vi "prueba_prueba.vi"() -> ()   [LabVIEW 2019]
uses:
  <vilib>/myRIO/Common/Instrument Driver Framework/myRIO v1.0/Encoder/typedefs/Encoder Signal Mode.ctl
  <vilib>/myRIO/Instrument Drivers/Onboard IO/Encoder/typedefs/Encoder Reference.ctl
  <vilib>/myRIO/Common/Instrument Driver Framework/Utilities/typedefs/myRIO Generic Hardware Reference.ctl
  <vilib>/myRIO/Common/Instrument Driver Framework/Utilities/typedefs/Hardware Version Enum.ctl
  <vilib>/myRIO/Common/Instrument Driver Framework/Utilities/typedefs/myRIO v1.0 Reference.ctl
  <vilib>/myRIO/Common/Instrument Driver Framework/Utilities/typedefs/Generic FPGA Reference.ctl
  <vilib>/myRIO/Common/Instrument Driver Framework/myRIO v1.0/Encoder/typedefs/Encoder Channels Enum.ctl
  <vilib>/myRIO/Common/Instrument Driver Framework/myRIO v1.0/Encoder/typedefs/Encoder Configuration v1.0.ctl
  <vilib>/userDefined/High Color/nirio_resource_hc.ctl
  <vilib>/myRIO/Instrument Drivers/Onboard IO/UART/typedef/VISA Configuration.ctl
  <vilib>/myRIO/Instrument Drivers/Onboard IO/DIO/typedefs/DIO Reference.ctl
  <vilib>/myRIO/Common/Instrument Driver Framework/myRIO v1.0/DIO/typedefs/DIO Channels List.ctl
  <vilib>/myRIO/Common/Instrument Driver Framework/myRIO v1.0/DIO/typedefs/DIO Channels Enum.ctl
  <vilib>/myRIO/Instrument Drivers/Onboard IO/PWM/typedefs/PWM Reference.ctl
  <vilib>/myRIO/Common/Instrument Driver Framework/myRIO v1.0/PWM/typedefs/PWM Channels Enum.ctl
  <vilib>/myRIO/Instrument Drivers/Onboard IO/PWM/typedefs/PWM Configuration.ctl
  <vilib>/myRIO/Common/Instrument Driver Framework/Utilities/vis/Is FPGA Ref Available.vi
  <vilib>/myRIO/Common/Instrument Driver Framework/myRIO v1.0/Encoder/vis/myRIO v1.1 Open Encoder.vi
  <vilib>/myRIO/Instrument Drivers/Onboard IO/Encoder/vis/Read.vi
  <vilib>/myRIO/Common/Instrument Driver Framework/myRIO v1.0/DIO/vis/myRIO v1.1 Open DIO.vi
  <vilib>/myRIO/Instrument Drivers/Onboard IO/DIO/vis/Write.vi
  <vilib>/myRIO/Common/Instrument Driver Framework/myRIO v1.0/PWM/vis/myRIO v1.1 Open PWM.vi
  <vilib>/myRIO/Instrument Drivers/Onboard IO/PWM/vis/Set Duty Cycle and Frequency.vi
  <vilib>/myRIO/Common/Instrument Driver Framework/Utilities/vis/Validate Channels.vi
  <vilib>/myRIO/Common/Instrument Driver Framework/myRIO v1.0/Encoder/vis/myRIO v1.0 Reserve Encoder.vi
  <vilib>/myRIO/Common/Instrument Driver Framework/myRIO v1.0/DIO/vis/myRIO v1.0 Reserve DIO.vi
  <vilib>/myRIO/Common/Instrument Driver Framework/myRIO v1.0/PWM/vis/myRIO v1.0 Reserve PWM.vi
  <vilib>/myRIO/Common/Instrument Driver Framework/myRIO v1.0/Encoder/vis/myRIO v1.0 Build MUX Configuration Encoder.vi
  <vilib>/myRIO/Common/Instrument Driver Framework/myRIO v1.0/Resource Manager/vis/myRIO v1.0 Reserve Channel List.vi
  <vilib>/myRIO/Common/Instrument Driver Framework/myRIO v1.0/DIO/vis/myRIO v1.0 Build MUX Configuration DIO.vi
  <vilib>/myRIO/Common/Instrument Driver Framework/myRIO v1.0/PWM/vis/myRIO v1.0 Build MUX Configuration PWM.vi
  <vilib>/myRIO/Common/Instrument Driver Framework/myRIO v1.0/Resource Manager/vis/myRIO v1.0 Create Configuration List.vi
  <vilib>/myRIO/Common/Instrument Driver Framework/myRIO v1.0/Resource Manager/vis/myRIO v1.0 Reserve Channel.vi
  <vilib>/myRIO/Common/Instrument Driver Framework/myRIO v1.0/Resource Manager/vis/myRIO v1.0 Unreserve Channel.vi
  <vilib>/myRIO/Common/Instrument Driver Framework/myRIO v1.0/Resource Manager/vis/myRIO v1.0 Build Mutex Name.vi
  <vilib>/Utility/VariantDataType/GetNumericInfo.vi
  <vilib>/Utility/error.llb/Error Cluster From Error Code.vi
  <vilib>/myRIO/Common/Instrument Driver Framework/myRIO v1.0/myRIO v1.1 Open.vi
  <vilib>/myRIO/Common/Instrument Driver Framework/Utilities/vis/IO Manager.vi
  <vilib>/myRIO/Common/Instrument Driver Framework/Utilities/vis/Configuration Manager.vi
  <vilib>/myRIO/Common/Instrument Driver Framework/myRIO v1.0/Resource Manager/vis/myRIO v1.0 Configure IO.vi
  <vilib>/myRIO/Common/Instrument Driver Framework/myRIO v1.0/myRIO v1.0 Close.vi
  <vilib>/myRIO/Common/Instrument Driver Framework/myRIO v1.0/Encoder/vis/myRIO v1.0 Configure Encoder.vi
  <vilib>/myRIO/Common/Instrument Driver Framework/myRIO v1.0/Encoder/vis/myRIO v1.0 Read Encoder.vi
  <vilib>/Instr/_visa.llb/VISA Configure Serial Port (Instr).vi
  <vilib>/express/express shared/transition.llb/Dynamic To Waveform Array.vi
  <vilib>/express/express signal manip/GetorSetDDTAttributes/Set DDT Attributes/SetT0.vi
  <vilib>/express/express shared/transition.llb/Waveform Array To Dynamic.vi
  <vilib>/myRIO/Common/Instrument Driver Framework/myRIO v1.0/DIO/vis/myRIO v1.0 Write DIO.vi
  <vilib>/myRIO/Common/Instrument Driver Framework/myRIO v1.0/PWM/vis/myRIO v1.0 Write PWM.vi
  <vilib>/myRIO/Express VI/Onboard IO/Encoder/Encoder Express VI.xnode
  <vilib>/myRIO/Instrument Drivers/Onboard IO/Encoder/vis/myRIO Encoder Open.xnode
  <vilib>/myRIO/Common/Instrument Driver Framework/myRIO v1.0/Encoder/typedefs/Encoder Count Direction Enum.ctl
  <vilib>/myRIO/Express VI/Onboard IO/UART/UART Express VI.xnode
  <vilib>/express/express signal manip/GetorSetDDTAttributes/Set DDT Attributes/Set DDT Properties.xnode
  <vilib>/myRIO/Express VI/Onboard IO/DO/DO Express VI.xnode
  <vilib>/myRIO/Instrument Drivers/Onboard IO/DIO/vis/myRIO DIO Open.xnode
  <vilib>/myRIO/Express VI/Onboard IO/PWM/PWM Express VI.xnode
  <vilib>/myRIO/Instrument Drivers/Onboard IO/PWM/vis/myRIO PWM Open.xnode
  <vilib>/myRIO/Instrument Drivers/Onboard IO/Encoder/Encoder.lvlib
  <vilib>/myRIO/Instrument Drivers/Onboard IO/PWM/PWM.lvlib
  <vilib>/myRIO/Instrument Drivers/Onboard IO/DIO/DIO.lvlib
  <vilib>/myRIO/Instrument Drivers/Onboard IO/UART/UART.lvlib
panel:
  out "Actividad B&P":dbl
  out "Actividad UAV":dbl
  in  "Cargar":bool
  out "Se mando caracteres?":bool
  out "Hay caracteres?":bool
  out "Posicion X vs Y":cluster{dbl[], dbl[]}(graph)
  out "Pitch":dbl(graph)
  out "Roll":dbl(graph)
  in  "B&P y UAV":string
  in  "Tab Control":T1(tab)
  out "PROGRESO DE SECUENCIA":dbl(slide) scale=0.0..100.0
  out "Tramo Actual":dbl
  out "Secuencia Activa":string
  out "Estado de Operacion":string
  out "POSICIÓN X":dbl
  out "POSICIÓN Y":dbl
  out "ORIENTACIÓN":dbl
  in  "Reiniciar_Ejecucion":bool
  in  "Iniciar_Secuencia":bool
  in  "Cargar_Secuencia":bool
  out "Tabla de secuencia":string[][](table)
  in  "Secuencia seleccionada":T2(ring)
  in  "RESET_TRAYECTO":bool
  out "Grafica_Velocidades_m_s":cluster{"Vel_Izq":dbl, "Vel_Der":dbl}(graph)
  out "Grafica_PWM_pct":T3(graph)
  out "Grafica_Trayectoria_XY":cluster{"t":dbl[], "t":dbl[]}(graph)
  in  "Velocidad Objetivo (m/s)":dbl
  in  "Duty Manual (%)":dbl
  in  "Distancia Objetivo (m)":dbl
  in  "Kp izquierda":dbl
  in  "Ki izquierda":dbl
  in  "Kp derecha":dbl
  in  "Ki derecha":dbl
  in  "Habilitar control Pi":bool
  in  "X Objetivo (metros)":dbl
  in  "Y Objetivo (metros)":dbl
  in  "Finalizar tramo (simulación)":bool
  out "Estado de máquina":T4(ring)
  out "Error de distancia (m)":dbl
  out "Error XY (m)":dbl
  out "Error angular (rad)":dbl
  out "Encoder izquierdo":i32
  out "Encoder derecho":i32
  out "Objetivo Alcanzado":bool
  out "PWM_Aplicado_Der_pct":dbl
  out "PWM_Aplicado_Izq_pct":dbl
  out "Distancia_Recorrida_m":dbl
  in  "Movimiento":T5(ring)
  out "Velocidad_Der_m_s":dbl
  out "Velocidad_Izq_m_s":dbl
  in  "STOP_GENERAL":bool
  # "DSM | ROBOT CONTROL CENTER"
  # "NI myRIO | Control y supervisión de base móvil"
  # "ESTADO DEL SISTEMA"
  # "Avance de la rutina"
  # "Secuencia pendiente de ejecucción"
  # "POSICIÓN ACTUAL DEL ROBOT"
  # "metros"
  # "metros"
  # "radianes"
  # "GESTOR DE SECUENCIAS"
  # "Selección, visualización y preparación de rutinas predefinidas"
  # "CONTROL DE SECUENCIA"
  # "SELECCIÓN DE RUTINA"
  # "MOVIMIENTOS PROGRAMADOS"
  # "Carga la rutina antes de iniciar su ejecución simulada."
  # "INTRUCCIONES DE USO"
  # "1. Selecciona una rutina. 2. Carga la secuencia. 3. Inicia la simulación. 4. Supervisa su progreso en OPERACION y DIAGNOSTICO."
  # "PARÁMETROS DE CONTROL"
  # "Configuración del movimiento y reguladores PI"
  # "MOVIMIENTO"
  # "REGULADORES PI"
  # "DESTINO XY"
  # "Coordenada objetivo respecto al origen de odometría"
  # "DIAGNÓSTICO DEL SISTEMA"
  # "Supervisión de estados, errores y sensores"
  # "MÁQUINA DE ESTADOS"
  # "ENCODERS"
  # "ERRORES DE CONTROL"
  # "-----------------------------------------"
  # "-----------------------------------------"
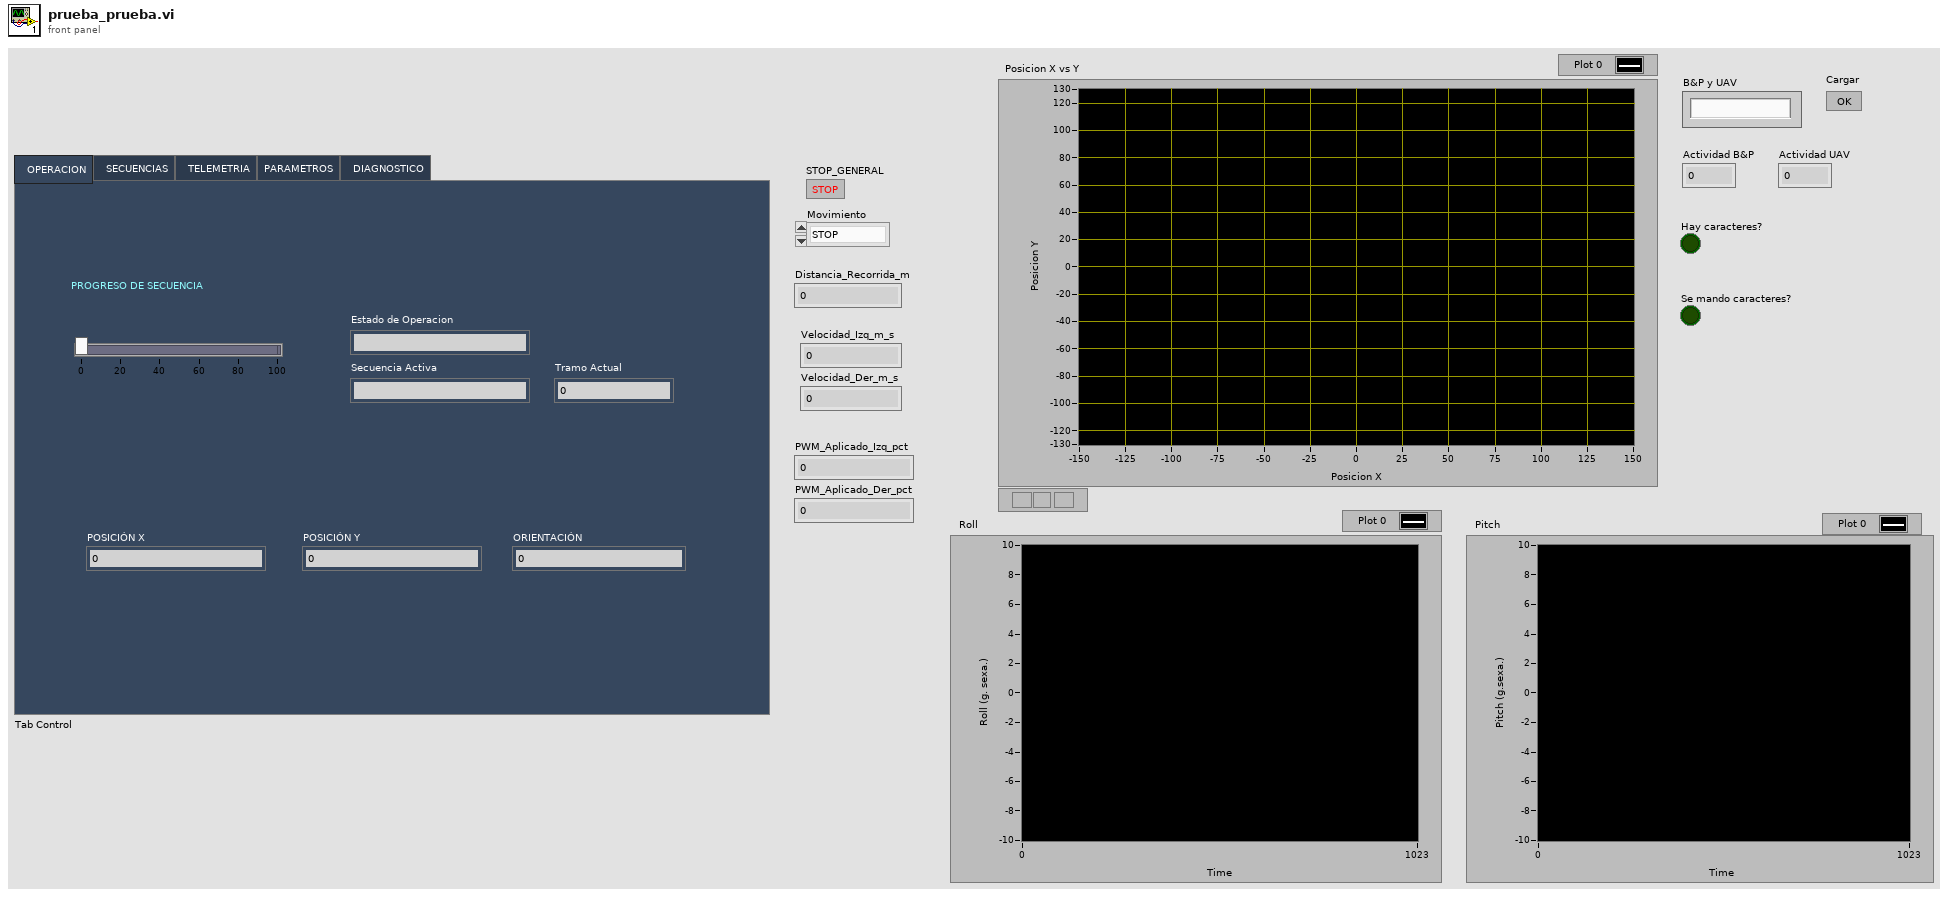
[diagram p1: front panel]
types:
  T1 = enum32{"\tOPERACION", "\tSECUENCIAS", "\tTELEMETRIA", "PARAMETROS", "\tDIAGNOSTICO"}
  T2 = enum16{"NINGUNA", "S1 - AVANCE Y RETORNO", "S2 - RECORRIDO EN L", "S3 - GIRO ACUMULADO", "S4 - DESTINO XY", "S5 - RAMPA 10 GRADOS"}
  T3 = cluster{"PWM_Final_Izq_pct":dbl, "PWM_Final_Der_pct":dbl}
  T4 = enum16{"ESPERA", "PREPARAR_TRAMO", "MOVER", "FRENAR", "COMPROBAR_LLEGADA", "SIGUIENTE_TRAMO", "FIN", "FALLO"}
  T5 = enum16{"STOP", "ADELANTE", "ATRÁS", "GIRO_IZQ", "GIRO_DER", "IR_A_XY"}
  T6 = typedef "UART.lvlib/VISA Configuration.ctl" = cluster{"baud rate (9600)":u32, "data bits (8)":u16, "parity (0:none)":enum16{"None", "Odd", "Even", "Mark", "Space"}, "stop bits (10: 1 bit)":u16, "flow control (0:none)":u16, "termination char\n(0xA = '\\n' = LF) ":u8, "Enable Termination\nChar (T)":bool, "timeout (10sec)":u32}
  T7 = typedef "DIO.lvlib/DIO Reference.ctl" = cluster{"myRIO Reference":T8, "DIO Channels List":T12}
  T8 = typedef "myRIO Generic Hardware Reference.ctl" = cluster{"myRIO Model":T9, "myRIO Hardware Reference":T10}
  T9 = typedef "Hardware Version Enum.ctl" = enum16{"Unknown", "myRIO-1900", "myRIO-1950", "roboRIO", "NI ELVIS RIO CM", "ELVIS III"}
  T10 = typedef "myRIO v1.0 Reference.ctl" = cluster{"Generic FPGA Reference":T11, "Allow multiple opens":bool}
  T11 = typedef "Generic FPGA Reference.ctl" = refnum<k20>
  T12 = typedef "DIO Channels List.ctl" = T13[]
  T13 = typedef "DIO Channels Enum.ctl" = enum16{"Not Connected", "C/DIO0", "C/DIO1", "C/DIO2", "C/DIO3", "C/DIO4", "C/DIO5", "C/DIO6", "C/DIO7", "A/DIO0", "A/DIO1", "A/DIO2", "A/DIO3", "A/DIO4", "A/DIO5", "A/DIO6", "A/DIO7", "A/DIO8", "A/DIO9", "A/DIO10", "A/DIO11", "A/DIO12", "A/DIO13", "A/DIO14", "A/DIO15", "A/DIO16", "A/DIO17", "A/DIO18", "A/DIO19", "B/DIO0", "B/DIO1", "B/DIO2", "B/DIO3", "B/DIO4", "B/DIO5", "B/DIO6", "B/DIO7", "B/DIO8", "B/DIO9", "B/DIO10", "B/DIO11", "B/DIO12", "B/DIO13", "B/DIO14", "B/DIO15", "B/DIO16", "B/DIO17", "B/DIO18", "B/DIO19", "LED0", "LED1", "LED2", "LED3", "Button0", "DIO/DIO0", "DIO/DIO1", "DIO/DIO2", "DIO/DIO3", "DIO/DIO4", "DIO/DIO5", "DIO/DIO6", "DIO/DIO7", "DIO/DIO8", "DIO/DIO9", "SPI/CS0", "SPI/CS1", "SPI/CS2", "SPI/CS3", "LED RADIO (Green)", "LED RADIO (Red)", "LED COMM (Green)", "LED COMM (Red)", "LED MODE (Green)", "LED MODE (Red)"}
  T14 = typedef "nirio_resource_hc.ctl" = tag
  T15 = typedef "PWM.lvlib/PWM Reference.ctl" = cluster{"myRIO Reference":T8, "PWM Channels Enum":T16, "PWM Configuration":T17}
  T16 = typedef "PWM Channels Enum.ctl" = enum16{"Not Connected", "C/PWM0", "C/PWM1", "A/PWM0", "A/PWM1", "A/PWM2", "A/PWM3", "A/PWM4", "A/PWM5", "A/PWM6", "A/PWM7", "A/PWM8", "A/PWM9", "A/PWM10", "A/PWM11", "A/PWM12", "A/PWM13", "A/PWM14", "A/PWM15", "A/PWM16", "A/PWM17", "A/PWM18", "A/PWM19", "B/PWM0", "B/PWM1", "B/PWM2", "B/PWM3", "B/PWM4", "B/PWM5", "B/PWM6", "B/PWM7", "B/PWM8", "B/PWM9", "B/PWM10", "B/PWM11", "B/PWM12", "B/PWM13", "B/PWM14", "B/PWM15", "B/PWM16", "B/PWM17", "B/PWM18", "B/PWM19", "PWM/PWM0", "PWM/PWM1", "PWM/PWM2", "PWM/PWM3", "PWM/PWM4", "PWM/PWM5", "PWM/PWM6", "PWM/PWM7", "PWM/PWM8", "PWM/PWM9"}
  T17 = typedef "PWM.lvlib/PWM Configuration.ctl" = cluster{"Frequency":dbl, "Duty Cycle":dbl}
  T18 = typedef "Encoder.lvlib/Encoder Reference.ctl" = cluster{"myRIO Reference":T8, "Encoder Channels Enum":T19}
  T19 = typedef "Encoder Channels Enum.ctl" = enum16{"Not Connected", "C/ENC0", "C/ENC1", "A/ENC", "A/ENC0", "A/ENC1", "A/ENC2", "A/ENC3", "A/ENC4", "A/ENC5", "A/ENC6", "A/ENC7", "A/ENC8", "A/ENC9", "B/ENC", "B/ENC0", "B/ENC1", "B/ENC2", "B/ENC3", "B/ENC4", "B/ENC5", "B/ENC6", "B/ENC7", "B/ENC8", "B/ENC9", "DIO/ENC0", "DIO/ENC1", "DIO/ENC2", "DIO/ENC3", "DIO/ENC4"}
  T20 = typedef "Encoder Signal Mode.ctl" = enum16{"Quadrature phase signal", "Step and direction signal"}
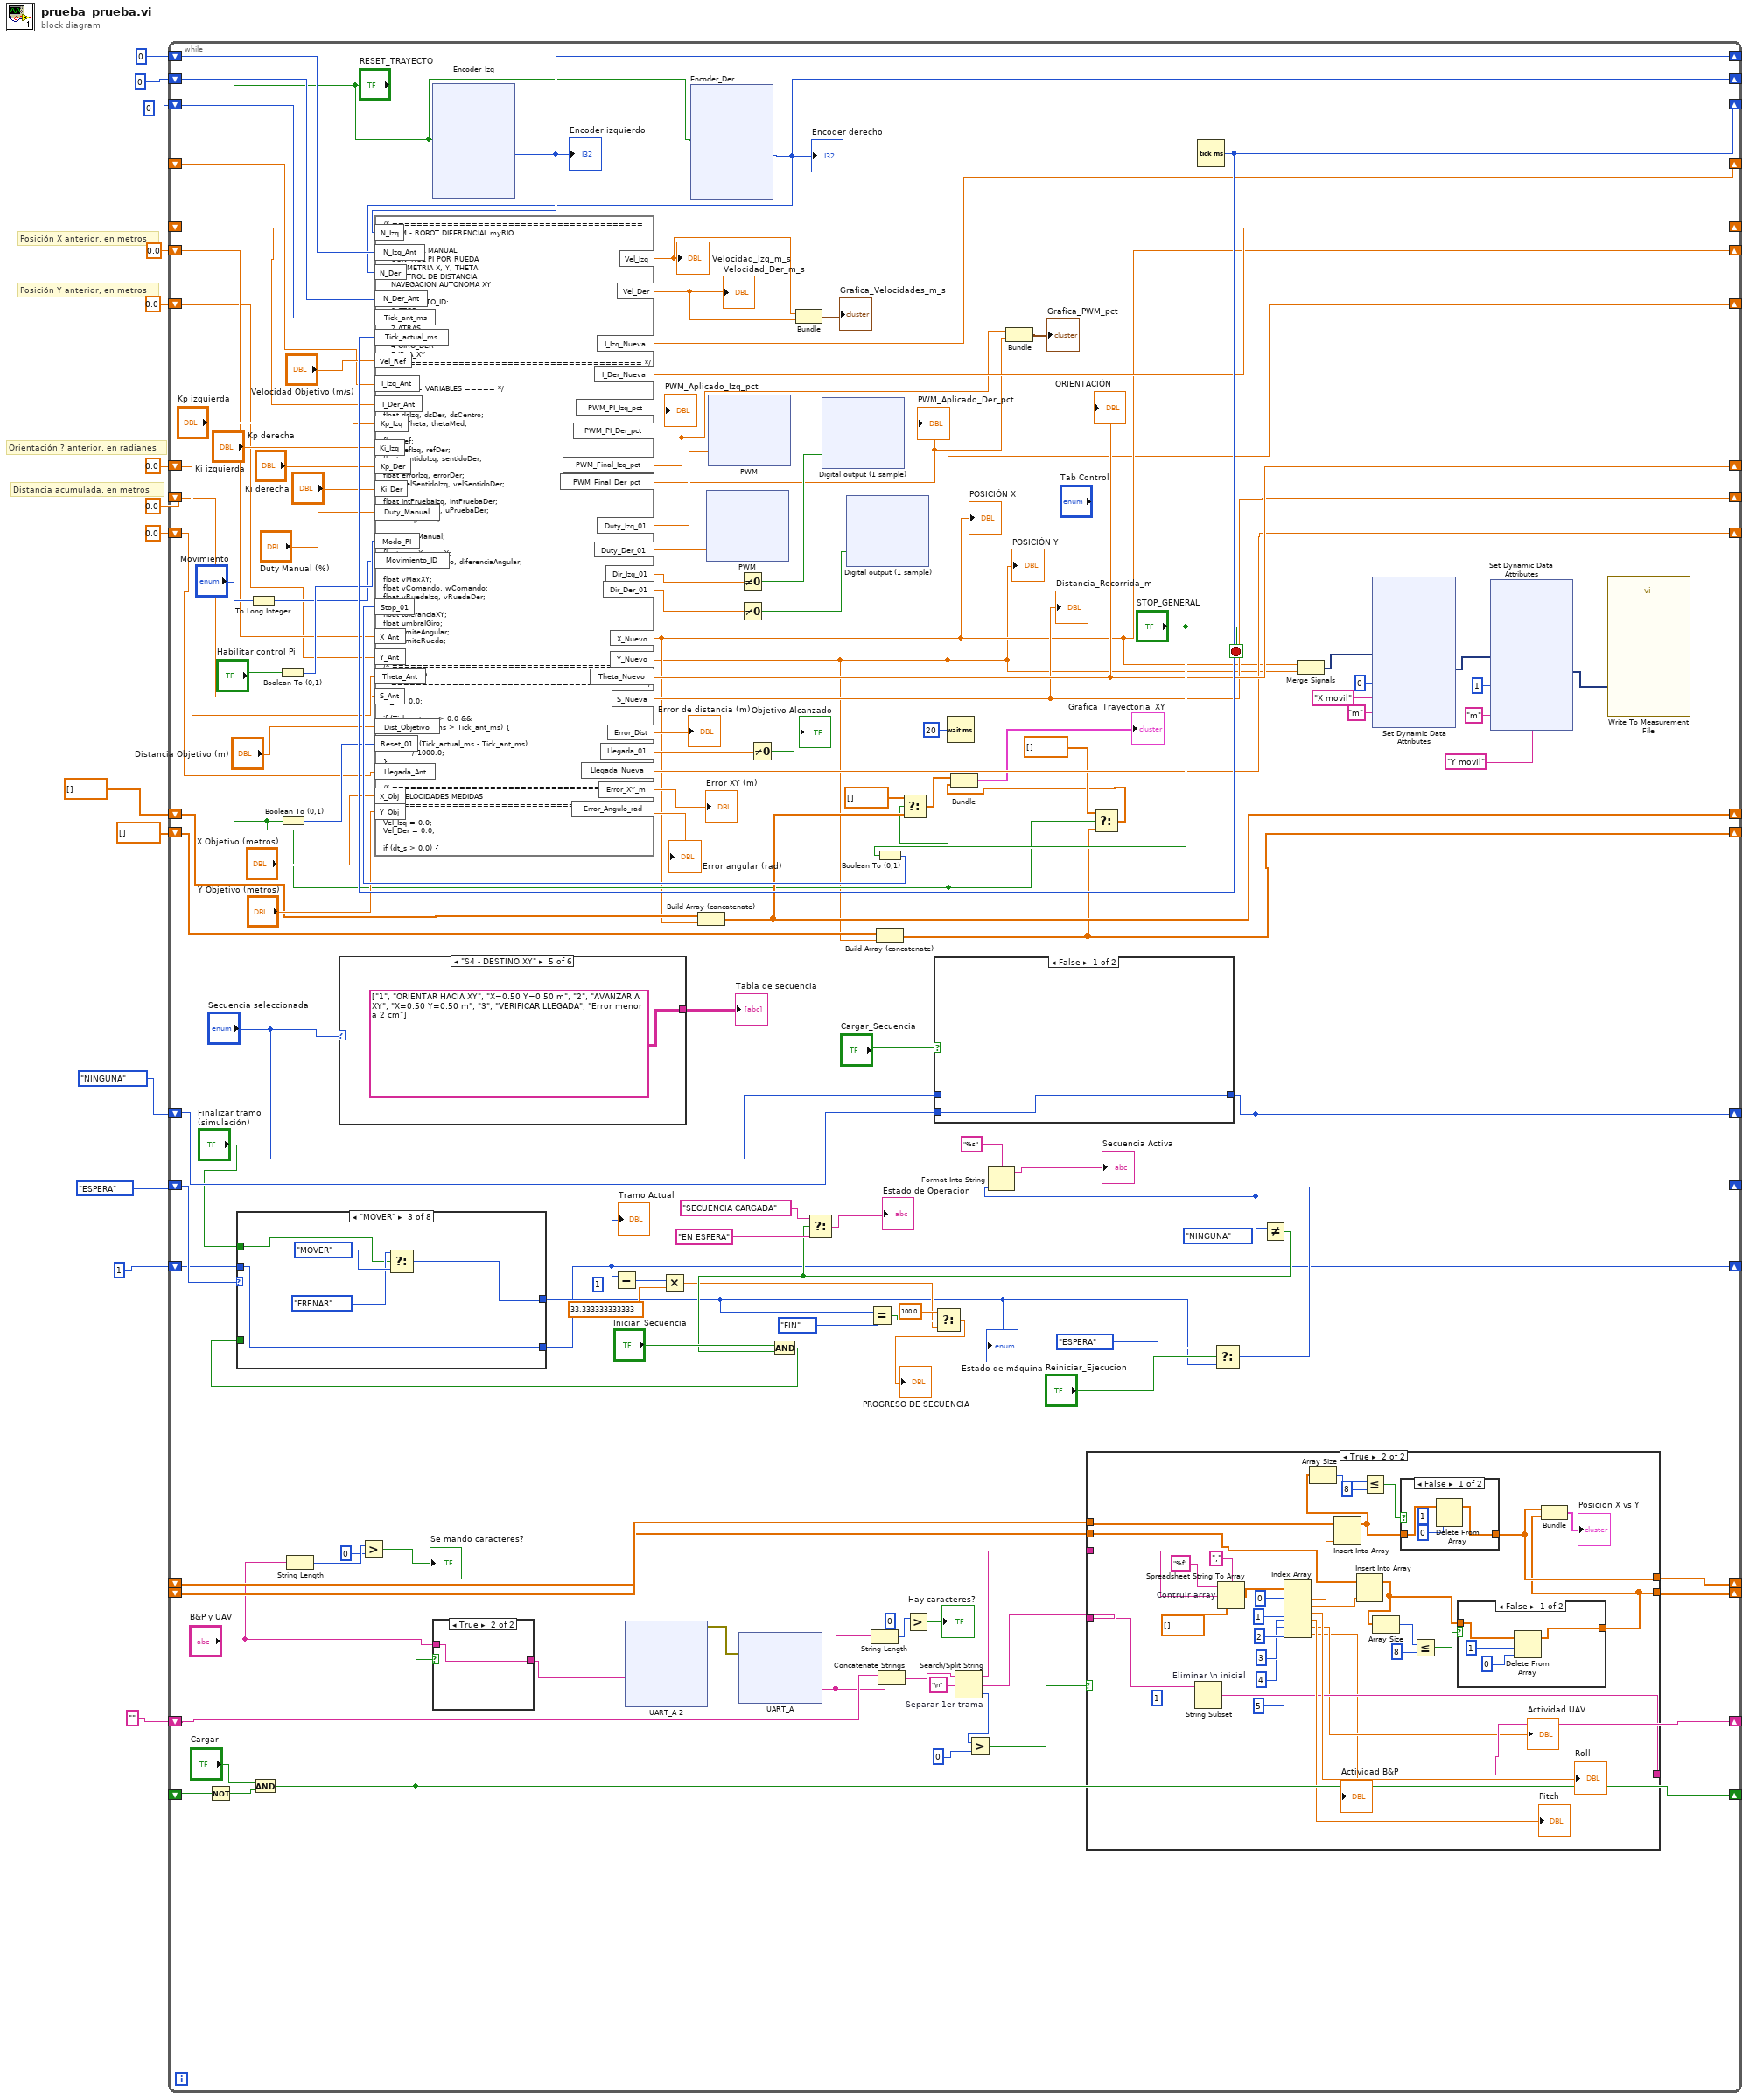
[diagram p0: block diagram]
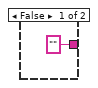
[diagram p2: hidden frame]
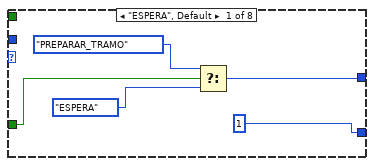
[diagram p6: hidden frame]
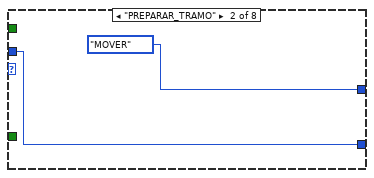
[diagram p7: hidden frame]
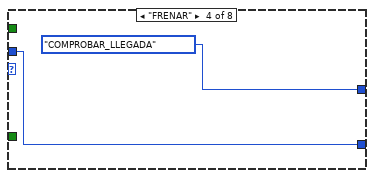
[diagram p8: hidden frame]
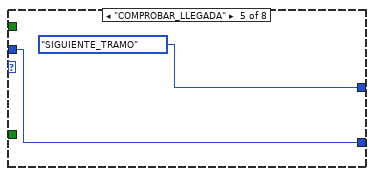
[diagram p9: hidden frame]
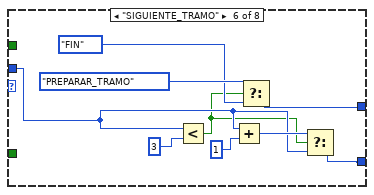
[diagram p10: hidden frame]
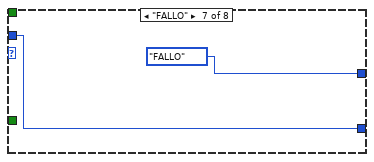
[diagram p11: hidden frame]
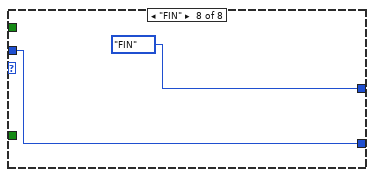
[diagram p12: hidden frame]
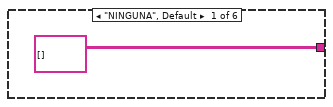
[diagram p14: hidden frame]
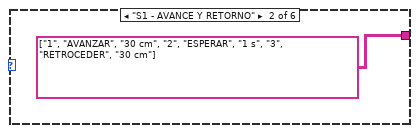
[diagram p15: hidden frame]
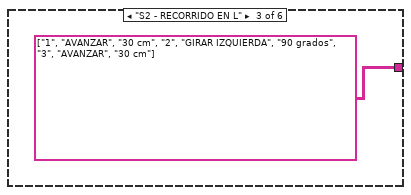
[diagram p16: hidden frame]
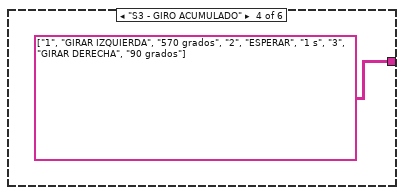
[diagram p17: hidden frame]
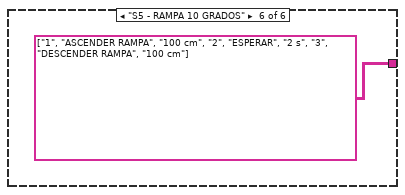
[diagram p18: hidden frame]
diagram:
  # "Distancia acumulada, en metros"
  # "Orientación ? anterior, en radianes"
  # "Posición Y anterior, en metros"
  # "Posición X anterior, en metros"
  n1 = while {
    shift-right: [w143] -> _
    shift-left: 0 ("Counter Value") -> [w142]
    shift-right: [w141] -> _
    shift-left: 0 ("Counter Value") -> [w140]
    shift-right: [w138] -> _
    shift-left: u32 0 ("millisecond timer value") -> [w139]
    shift-right: [w132] -> _
    shift-left: _ -> [w133]
    shift-right: [w130] -> _
    shift-left: _ -> [w131]
    shift-right: [w25] -> _
    shift-left: 0.0 ("X_Nuevo") -> [w116]
    shift-right: [w24] -> _
    shift-left: 0.0 ("Y_Nuevo") -> [w115]
    shift-right: [w113] -> _
    shift-left: 0.0 ("Theta_Nuevo") -> [w114]
    shift-right: [w111] -> _
    shift-left: 0.0 ("S_Nueva") -> [w112]
    shift-right: [w104] -> _
    shift-left: 0.0 ("Llegada_Nueva") -> [w103]
    shift-right: [w90] -> _
    shift-left: dbl[] [] -> [w92]
    shift-right: [w89] -> _
    shift-left: dbl[] [] -> [w91]
    shift-right: [w77] -> _
    shift-left: T2."NINGUNA" ("Seleccion_Secuencia") -> [w80]
    shift-right: [w56] -> _
    shift-left: T4."ESPERA" -> [w72]
    shift-right: [w54] -> _
    shift-left: 1 -> [w67]
    shift-right: [w45] -> _
    shift-left: "" -> [w48]
    shift-right: [w42] -> _
    shift-left: _ -> [w43]
    shift-right: [w41] -> _
    shift-left: _ -> [w40]
    shift-right: [w27] -> _
    shift-left: _ -> [w26]
    stop <- "STOP_GENERAL" stop-if-true
    n2 = Not(x=w26) -> (.not. x?=w28:bool)
    n3 = To Long Integer(number="Movimiento") -> (32bit integer=w124:i32)
    n4 = And(x="Cargar", y=w28) -> (x .and. y?=w27:bool)
    n5 = Boolean To (0,1)(Boolean="Habilitar control Pi") -> (0, 1=w134:i16)
    n6 = Boolean To (0,1)(Boolean="RESET_TRAYECTO") -> (0, 1=w109:i16)
    n7 = String Length(string="B&P y UAV") -> (length=w34:i32)
    n8 = case shown="\"S4 - DESTINO XY\"" "Secuencia seleccionada" {
      tunnel: [string[][] [] ("Tabla_Secuencia") string[][] [["1", "AVANZAR", "30 cm"], ["2", "ESPERAR", "1 s"], ["3", "RETROCEDER", "30 cm"]] ("Tabla_Secuencia") string[][] [["1", "AVANZAR", "30 cm"], ["2", "GIRAR IZQUIERDA", "90 grados"], ["3", "AVANZAR", "30 cm"]] ("Tabla_Secuencia") string[][] [["1", "GIRAR IZQUIERDA", "570 grados"], ["2", "ESPERAR", "1 s"], ["3", "GIRAR DERECHA", "90 grados"]] ("Tabla_Secuencia") string[][] [["1", "ORIENTAR HACIA XY", "X=0.50 Y=0.50 m"], ["2", "AVANZAR A XY", "X=0.50 Y=0.50 m"], ["3", "VERIFICAR LLEGADA", "Error menor a 2 cm"]] ("Tabla_Secuencia") string[][] [["1", "ASCENDER RAMPA", "100 cm"], ["2", "ESPERAR", "2 s"], ["3", "DESCENDER RAMPA", "100 cm"]] ("Tabla_Secuencia")] -> w83
      frame "NINGUNA", Default {
      }
      frame "S1 - AVANCE Y RETORNO" {
      }
      frame "S2 - RECORRIDO EN L" {
      }
      frame "S3 - GIRO ACUMULADO" {
      }
      frame "S4 - DESTINO XY" {
      }
      frame "S5 - RAMPA 10 GRADOS" {
      }
    }
    "Tabla de secuencia" <- w83
    n9 = Greater?(x=w34, y=0) -> (0:→"Se mando caracteres?":bool)
    n10 = xnode "Encoder_Izq"("Reset Counter"="RESET_TRAYECTO") -> ("Counter Value"=w143:i32)  [unwired: 1 in, 3 out]
    "Encoder izquierdo" <- w143
    n11 = case shown="True" w27 {
      tunnel: "B&P y UAV" -> [_ w180]
      tunnel: ["" ("B&P y UAV") w180] -> w30
      frame False {
      }
      frame True {
      }
    }
    n12 = xnode "UART_A 2"("Characters to Write"=w30) -> ("error out"=w53:errorcluster)  [unwired: 1 in, 1 out]
    n13 = xnode "Encoder_Der"("Reset Counter"="RESET_TRAYECTO") -> ("Counter Value"=w141:i32)  [unwired: 1 in, 3 out]
    "Encoder derecho" <- w141
    n14 = xnode "UART_A"("error in (no error)"=w53) -> ("Characters Read"=w39:string)  [unwired: 1 out]
    n15 = String Length(string=w39) -> (length=w38:i32)
    n16 = Boolean To (0,1)(Boolean="STOP_GENERAL") -> (0, 1=w117:i16)
    n17 = Concatenate Strings(w48, w39) -> (w51:string)
    n18 = Greater?(x=w38, y=0) -> (0:→"Hay caracteres?":bool)
    n19 = case shown="False" "Cargar_Secuencia" {
      tunnel: "Secuencia seleccionada" -> [_ w290]
      tunnel: [w289 w290] -> w77
      tunnel: w80 -> [w289 _]
      frame False {
      }
      frame True {
      }
    }
    n20 = Wait (ms)(milliseconds to wait=u32 20) -> ()  [unwired: 1 out]
    n21 = Search/Split String "Separar 1er trama"(string=w51, search string/char (-)="\n") -> (substring before match=w46:string, match + rest of string=w47:string, offset of match=w49:i32)  [unwired: 1 in]
    n22 = Greater?(x=w49, y=0) -> (0:w35:bool)
    n23 = Format Into String(format string="%s", w77) -> (resulting string=→"Secuencia Activa":string)  [unwired: 2 in, 1 out]
    n24 = case shown="True" w35 {
      tunnel: w47 -> [_ w208]
      tunnel: w46 -> [w183 w209]
      tunnel: [w183 w207] -> w45
      tunnel: w43 -> [w181 w202]
      tunnel: [w181 w197] -> w42
      tunnel: [w182 w188] -> w41
      tunnel: w40 -> [w182 w201]
      frame False {
      }
      frame True {
        n25 = String Subset "Eliminar \\n inicial"(string=w208, offset (0)=1) -> (substring=w207:string)  [unwired: 1 in]
        n26 = Spreadsheet String To Array "Contruir array"(delimiter (Tab)=",", format string="%f", spreadsheet string=w209, array type (2D Dbl)=dbl[] []) -> (array=w216:dbl[])
        n27 = Index Array(array=w216, index #1=0 ("index"), index #2=1 ("index"), index #3=2 ("index"), index #4=3 ("index"), index #5=4 ("index"), index #6=5 ("index")) -> (element #1=w199:dbl, element #2=w198:dbl, element #3=→"Roll":dbl, element #4=→"Pitch":dbl, element #5=→"Actividad UAV":dbl, element #6=→"Actividad B&P":dbl)
        n28 = Insert Into Array(array=w202, new element=w199) -> (w196:dbl[])  [unwired: 1 in]
        n29 = Array Size(array=w196) -> (size(s)=w195:i32)
        n30 = Insert Into Array(array=w201, new element=w198) -> (w189:dbl[])  [unwired: 1 in]
        n31 = Less Or Equal?(x=w195, y=8) -> (x <= y?=w193:bool)
        n32 = Array Size(array=w189) -> (size(s)=w192:i32)
        n33 = case shown="False" w193 {
          tunnel: w196 -> [w225 w226]
          tunnel: [w222 w226] -> w197
          frame False {
            n34 = Delete From Array(array=w225, length=1, index=0) -> (array with subset deleted=w222:dbl[])  [unwired: 1 out]
          }
          frame True {
          }
        }
        n35 = Less Or Equal?(x=w192, y=8) -> (x <= y?=w190:bool)
        n36 = case shown="False" w190 {
          tunnel: w189 -> [w220 w221]
          tunnel: [w217 w221] -> w188
          frame False {
            n37 = Delete From Array(array=w220, length=1, index=0) -> (array with subset deleted=w217:dbl[])  [unwired: 1 out]
          }
          frame True {
          }
        }
        n38 = Bundle(w197, w188) -> (→"Posicion X vs Y":cluster{dbl[], dbl[]})  [unwired: 1 in]
      }
    }
    n39 = Tick Count (ms)() -> (millisecond timer value=w138:u32)
    n40 = formula code="/* =========================================\n   DSM - ROBOT DIFERENCIAL myRIO\n\n   CONTROL MANUAL\n   CONTROL PI POR RUEDA\n   ODOMETRIA X, Y, THETA\n   CONTROL DE DISTANCIA\n   NAVEGACION AUTONOMA XY\n\n   MOVIMIENTO_ID:\n   0 STOP\n   1 ADELANTE\n   2 ATRAS\n   3 GIRO_IZQ\n   4 GIRO_DER\n   5 IR_A_XY\n   ========================================= */\n\n\n/* ===== VARIABLES ===== */\n\nfloat dt_s;\nfloat dsIzq, dsDer, dsCentro;\nfloat dTheta, thetaMed;\n\nfloat ref;\nfloat refIzq, refDer;\nfloat sentidoIzq, sentidoDer;\n\nfloat errorIzq, errorDer;\nfloat velSentidoIzq, velSentidoDer;\n\nfloat intPruebaIzq, intPruebaDer;\nfloat uPruebaIzq, uPruebaDer;\nfloat uIzq, uDer;\n\nfloat dutyManual;\n\nfloat errorX, errorY;\nfloat anguloObjetivo, diferenciaAngular;\n\nfloat vMaxXY;\nfloat vComando, wComando;\nfloat vRuedaIzq, vRuedaDer;\n\nfloat toleranciaXY;\nfloat umbralGiro;\nfloat limiteAngular;\nfloat limiteRueda;\n\n\n/* =========================================\n   1. TIEMPO\n   ========================================= */\n\ndt_s = 0.0;\n\nif (Tick_ant_ms > 0.0 &&\n    Tick_actual_ms > Tick_ant_ms) {\n\n    dt_s = (Tick_actual_ms - Tick_ant_ms)\n           / 1000.0;\n}\n\n\n/* =========================================\n   2. VELOCIDADES MEDIDAS\n   ========================================= */\n\nVel_Izq = 0.0;\nVel_Der = 0.0;\n\nif (dt_s > 0.0) {\n\n    Vel_Izq = (N_Izq - N_Izq_Ant)\n              * 0.0002151 / dt_s;\n\n    Vel_Der = (N_Der - N_Der_Ant)\n              * (-0.0002151) / dt_s;\n}\n\n\n/* =========================================\n   3. ODOMETRIA\n   ========================================= */\n\nX_Nuevo = X_Ant;\nY_Nuevo = Y_Ant;\nTheta_Nuevo = Theta_Ant;\nS_Nueva = S_Ant;\n\nif (dt_s > 0.0) {\n\n    dsIzq = (N_Izq - N_Izq_Ant)\n             * 0.0002151;\n\n    dsDer = (N_Der - N_Der_Ant)\n             * (-0.0002151);\n\n    dsCentro = (dsIzq + dsDer) / 2.0;\n\n    dTheta = (dsDer - dsIzq) / 0.3794;\n\n    thetaMed = Theta_Ant + dTheta / 2.0;\n\n    X_Nuevo = X_Ant\n            + dsCentro * cos(thetaMed);\n\n    Y_Nuevo = Y_Ant\n            + dsCentro * sin(thetaMed);\n\n    Theta_Nuevo = Theta_Ant + dTheta;\n\n    if (dsCentro >= 0.0) {\n        S_Nueva = S_Ant + dsCentro;\n    } else {\n        S_Nueva = S_Ant - dsCentro;\n    }\n}\n\n\n/* =========================================\n   4. RESET DE ODOMETRIA\n   ========================================= */\n\nif (Reset_01 == 1) {\n\n    X_Nuevo = 0.0;\n    Y_Nuevo = 0.0;\n\n    Theta_Nuevo = 0.0;\n    S_Nueva = 0.0;\n}\n\n\n/* =========================================\n   5. ERRORES DE TRAYECTORIA XY\n   ========================================= */\n\nerrorX = X_Obj - X_Nuevo;\nerrorY = Y_Obj - Y_Nuevo;\n\nError_XY_m = sqrt(errorX * errorX\n                + errorY * errorY);\n\nError_Angulo_rad = 0.0;\n\nif (Error_XY_m > 0.000001) {\n\n    anguloObjetivo = atan2(errorY, errorX);\n\n    diferenciaAngular =\n        anguloObjetivo - Theta_Nuevo;\n\n    Error_Angulo_rad =\n        atan2(sin(diferenciaAngular),\n              cos(diferenciaAngular));\n}\n\n\n/* =========================================\n   6. DISTANCIA Y MEMORIA DE LLEGADA\n   ========================================= */\n\nError_Dist = Dist_Objetivo - S_Nueva;\n\nLlegada_Nueva = Llegada_Ant;\n\ntoleranciaXY = 0.02;\n\n/* RESET borra la memoria de llegada */\n\nif (Reset_01 == 1) {\n\n    Llegada_Nueva = 0.0;\n\n} else {\n\n    /* Llegada por distancia */\n\n    if ((Movimiento_ID == 1 ||\n         Movimiento_ID == 2) &&\n        Dist_Objetivo > 0.0 &&\n        S_Nueva >= Dist_Objetivo) {\n\n        Llegada_Nueva = 1.0;\n    }\n\n    /* Llegada por posicion XY */\n\n    if (Movimiento_ID == 5 &&\n        Error_XY_m <= toleranciaXY) {\n\n        Llegada_Nueva = 1.0;\n    }\n}\n\nLlegada_01 = Llegada_Nueva;\n\n\n/* =========================================\n   7. REFERENCIA DE VELOCIDAD\n   ========================================= */\n\nref = Vel_Ref;\n\nif (ref < 0.0) {\n    ref = -ref;\n}\n\n/* Referencias iniciales */\n\nrefIzq = ref;\nrefDer = ref;\n\nsentidoIzq = 0.0;\nsentidoDer = 0.0;\n\n\n/* =========================================\n   8. MOVIMIENTOS CONVENCIONALES\n   ========================================= */\n\nif (Movimiento_ID == 1) {\n\n    sentidoIzq = 1.0;\n    sentidoDer = 1.0;\n}\n\nif (Movimiento_ID == 2) {\n\n    sentidoIzq = -1.0;\n    sentidoDer = -1.0;\n}\n\nif (Movimiento_ID == 3) {\n\n    sentidoIzq = -1.0;\n    sentidoDer = 1.0;\n}\n\nif (Movimiento_ID == 4) {\n\n    sentidoIzq = 1.0;\n    sentidoDer = -1.0;\n}\n\n\n/* =========================================\n   9. CONTROL DE TRAYECTORIA XY\n   ========================================= */\n\n/*\n   ESTE MODO NECESITA MODO_PI = 1.\n\n   VELOCIDAD MAXIMA XY:\n   0.05 m/s\n\n   VELOCIDAD ANGULAR MAXIMA:\n   0.20 rad/s\n\n   TOLERANCIA DE LLEGADA:\n   0.02 m\n*/\n\nif (Movimiento_ID == 5 &&\n    Modo_PI == 1 &&\n    Llegada_Nueva == 0.0 &&\n    ref > 0.0) {\n\n    /* Limitar velocidad por seguridad */\n\n    vMaxXY = ref;\n\n    if (vMaxXY > 0.05) {\n        vMaxXY = 0.05;\n    }\n\n    umbralGiro = 0.20;\n    limiteAngular = 0.20;\n    limiteRueda = 0.05;\n\n    vComando = 0.0;\n    wComando = 0.0;\n\n\n    /* ===== ORIENTAR EL ROBOT ===== */\n\n    if (Error_Angulo_rad > umbralGiro ||\n        Error_Angulo_rad < -umbralGiro) {\n\n        /* Primero girar sobre el eje */\n\n        vComando = 0.0;\n\n        wComando = 1.2 * Error_Angulo_rad;\n\n    } else {\n\n        /* ===== AVANZAR HACIA OBJETIVO ===== */\n\n        vComando = vMaxXY;\n\n        /* Reducir velocidad cerca del destino */\n\n        if (Error_XY_m < 0.08) {\n\n            vComando = 0.8 * Error_XY_m;\n\n            if (vComando < 0.025 &&\n                vMaxXY >= 0.025) {\n\n                vComando = 0.025;\n            }\n\n            if (vComando > vMaxXY) {\n                vComando = vMaxXY;\n            }\n        }\n\n        /* Corregir orientacion en movimiento */\n\n        wComando = 1.2 * Error_Angulo_rad;\n    }\n\n\n    /* Limitar velocidad angular */\n\n    if (wComando > limiteAngular) {\n        wComando = limiteAngular;\n    }\n\n    if (wComando < -limiteAngular) {\n        wComando = -limiteAngular;\n    }\n\n\n    /* =====================================\n       10. CINEMATICA DIFERENCIAL\n       ===================================== */\n\n    vRuedaIzq =\n        vComando - 0.1897 * wComando;\n\n    vRuedaDer =\n        vComando + 0.1897 * wComando;\n\n\n    /* Limitar referencia de rueda izquierda */\n\n    if (vRuedaIzq > limiteRueda) {\n        vRuedaIzq = limiteRueda;\n    }\n\n    if (vRuedaIzq < -limiteRueda) {\n        vRuedaIzq = -limiteRueda;\n    }\n\n\n    /* Limitar referencia de rueda derecha */\n\n    if (vRuedaDer > limiteRueda) {\n        vRuedaDer = limiteRueda;\n    }\n\n    if (vRuedaDer < -limiteRueda) {\n        vRuedaDer = -limiteRueda;\n    }\n\n\n    /* ===== SENTIDO RUEDA IZQUIERDA ===== */\n\n    sentidoIzq = 0.0;\n    refIzq = vRuedaIzq;\n\n    if (refIzq > 0.0) {\n        sentidoIzq = 1.0;\n    }\n\n    if (refIzq < 0.0) {\n        sentidoIzq = -1.0;\n        refIzq = -refIzq;\n    }\n\n\n    /* ===== SENTIDO RUEDA DERECHA ===== */\n\n    sentidoDer = 0.0;\n    refDer = vRuedaDer;\n\n    if (refDer > 0.0) {\n        sentidoDer = 1.0;\n    }\n\n    if (refDer < 0.0) {\n        sentidoDer = -1.0;\n        refDer = -refDer;\n    }\n}\n\n\n/* =========================================\n   11. INICIALIZAR SALIDAS\n   ========================================= */\n\nI_Izq_Nueva = 0.0;\nI_Der_Nueva = 0.0;\n\nPWM_PI_Izq_pct = 0.0;\nPWM_PI_Der_pct = 0.0;\n\nPWM_Final_Izq_pct = 0.0;\nPWM_Final_Der_pct = 0.0;\n\nDuty_Izq_01 = 0.0;\nDuty_Der_01 = 0.0;\n\nDir_Izq_01 = 0.0;\nDir_Der_01 = 0.0;\n\n\n/* =========================================\n   12. HABILITACION DEL MOVIMIENTO\n   ========================================= */\n\nif (Stop_01 == 0 &&\n    Reset_01 == 0 &&\n    Llegada_Nueva == 0.0 &&\n    (\n      (\n        Movimiento_ID >= 1 &&\n        Movimiento_ID <= 4 &&\n        (\n          Movimiento_ID >= 3 ||\n          Dist_Objetivo > 0.0\n        )\n      )\n      ||\n      (\n        Movimiento_ID == 5 &&\n        Modo_PI == 1 &&\n        ref > 0.0\n      )\n    )) {\n\n\n    /* =====================================\n       13. CONTROL PI POR RUEDA\n       ===================================== */\n\n    if (Modo_PI == 1 &&\n        dt_s > 0.0) {\n\n\n        /* ===== PI IZQUIERDO ===== */\n\n        if (sentidoIzq != 0.0 &&\n            refIzq > 0.0) {\n\n            velSentidoIzq =\n                Vel_Izq * sentidoIzq;\n\n            errorIzq =\n                refIzq - velSentidoIzq;\n\n            I_Izq_Nueva = I_Izq_Ant;\n\n            if (Ki_Izq > 0.0) {\n\n                intPruebaIzq =\n                    I_Izq_Ant\n                    + errorIzq * dt_s;\n\n                uPruebaIzq =\n                    Kp_Izq * errorIzq\n                    + Ki_Izq * intPruebaIzq;\n\n                if ((uPruebaIzq > 100.0 &&\n                     errorIzq > 0.0) ||\n                    (uPruebaIzq < 0.0 &&\n                     errorIzq < 0.0)) {\n\n                    I_Izq_Nueva = I_Izq_Ant;\n\n                } else {\n\n                    I_Izq_Nueva = intPruebaIzq;\n                }\n            }\n\n            uIzq =\n                Kp_Izq * errorIzq\n                + Ki_Izq * I_Izq_Nueva;\n\n            if (uIzq > 100.0) {\n                uIzq = 100.0;\n            }\n\n            if (uIzq < 0.0) {\n                uIzq = 0.0;\n            }\n\n            PWM_PI_Izq_pct =\n                sentidoIzq * uIzq;\n        }\n\n\n        /* ===== PI DERECHO ===== */\n\n        if (sentidoDer != 0.0 &&\n            refDer > 0.0) {\n\n            velSentidoDer =\n                Vel_Der * sentidoDer;\n\n            errorDer =\n                refDer - velSentidoDer;\n\n            I_Der_Nueva = I_Der_Ant;\n\n            if (Ki_Der > 0.0) {\n\n                intPruebaDer =\n                    I_Der_Ant\n                    + errorDer * dt_s;\n\n                uPruebaDer =\n                    Kp_Der * errorDer\n                    + Ki_Der * intPruebaDer;\n\n                if ((uPruebaDer > 100.0 &&\n                     errorDer > 0.0) ||\n                    (uPruebaDer < 0.0 &&\n                     errorDer < 0.0)) {\n\n                    I_Der_Nueva = I_Der_Ant;\n\n                } else {\n\n                    I_Der_Nueva = intPruebaDer;\n                }\n            }\n\n            uDer =\n                Kp_Der * errorDer\n                + Ki_Der * I_Der_Nueva;\n\n            if (uDer > 100.0) {\n                uDer = 100.0;\n            }\n\n            if (uDer < 0.0) {\n                uDer = 0.0;\n            }\n\n            PWM_PI_Der_pct =\n                sentidoDer * uDer;\n        }\n\n\n        /* PWM final controlado por PI */\n\n        PWM_Final_Izq_pct =\n            PWM_PI_Izq_pct;\n\n        PWM_Final_Der_pct =\n            PWM_PI_Der_pct;\n    }\n\n\n    /* =====================================\n       14. CONTROL MANUAL\n       ===================================== */\n\n    if (Modo_PI == 0) {\n\n        dutyManual = Duty_Manual;\n\n        if (dutyManual > 100.0) {\n            dutyManual = 100.0;\n        }\n\n        if (dutyManual < 0.0) {\n            dutyManual = 0.0;\n        }\n\n        PWM_Final_Izq_pct =\n            sentidoIzq * dutyManual;\n\n        PWM_Final_Der_pct =\n            sentidoDer * dutyManual;\n\n        /* Compensacion: solo ADELANTE manual, -5% rueda derecha */\n        if (Movimiento_ID == 1) {\n            PWM_Final_Der_pct = PWM_Final_Der_pct * 0.99;\n        }\n    }\n\n\n    /* =====================================\n       15. DIRECCIONES FISICAS CORREGIDAS\n       ===================================== */\n\n    Dir_Izq_01 = 0.0;\n\n    if (PWM_Final_Izq_pct < 0.0) {\n        Dir_Izq_01 = 1.0;\n    }\n\n    Dir_Der_01 = 0.0;\n\n    if (PWM_Final_Der_pct > 0.0) {\n        Dir_Der_01 = 1.0;\n    }\n\n\n    /* =====================================\n       16. NORMALIZAR PWM A 0..1\n       ===================================== */\n\n    Duty_Izq_01 = PWM_Final_Izq_pct;\n    Duty_Der_01 = PWM_Final_Der_pct;\n\n    if (Duty_Izq_01 < 0.0) {\n        Duty_Izq_01 = -Duty_Izq_01;\n    }\n\n    if (Duty_Der_01 < 0.0) {\n        Duty_Der_01 = -Duty_Der_01;\n    }\n\n    Duty_Izq_01 =\n        Duty_Izq_01 / 100.0;\n\n    Duty_Der_01 =\n        Duty_Der_01 / 100.0;\n}\n\n\n/* =========================================\n   17. RESET DE CONTROL Y SALIDAS\n   ========================================= */\n\nif (Reset_01 == 1) {\n\n    I_Izq_Nueva = 0.0;\n    I_Der_Nueva = 0.0;\n\n    PWM_PI_Izq_pct = 0.0;\n    PWM_PI_Der_pct = 0.0;\n\n    PWM_Final_Izq_pct = 0.0;\n    PWM_Final_Der_pct = 0.0;\n\n    Duty_Izq_01 = 0.0;\n    Duty_Der_01 = 0.0;\n\n    Dir_Izq_01 = 0.0;\n    Dir_Der_01 = 0.0;\n}"("N_Izq"=w143, "N_Izq_Ant"=w142, "N_Der"=w141, "N_Der_Ant"=w140, "Tick_ant_ms"=w139, "Tick_actual_ms"=w138, "Vel_Ref"="Velocidad Objetivo (m/s)", "I_Izq_Ant"=w133, "I_Der_Ant"=w131, "Kp_Izq"="Kp izquierda", "Ki_Izq"="Ki izquierda", "Kp_Der"="Kp derecha", "Ki_Der"="Ki derecha", "Duty_Manual"="Duty Manual (%)", "Modo_PI"=w134, "Movimiento_ID"=w124, "Stop_01"=w117, "X_Ant"=w116, "Y_Ant"=w115, "Theta_Ant"=w114, "S_Ant"=w112, "Dist_Objetivo"="Distancia Objetivo (m)", "Reset_01"=w109, "Llegada_Ant"=w103, "X_Obj"="X Objetivo (metros)", "Y_Obj"="Y Objetivo (metros)") -> ("Vel_Izq"=w97:dbl, "Vel_Der"=w96:dbl, "I_Izq_Nueva"=w132:dbl, "I_Der_Nueva"=w130:dbl, "PWM_Final_Izq_pct"=w94:dbl, "PWM_Final_Der_pct"=w93:dbl, "Duty_Izq_01"=w123:dbl, "Duty_Der_01"=w122:dbl, "Dir_Izq_01"=w121:dbl, "Dir_Der_01"=w119:dbl, "Y_Nuevo"=w24:dbl, "Theta_Nuevo"=w113:dbl, "S_Nueva"=w111:dbl, "X_Nuevo"=w25:dbl, "Error_Dist"=→"Error de distancia (m)":dbl, "Llegada_01"=w107:dbl, "Llegada_Nueva"=w104:dbl, "Error_XY_m"=→"Error XY (m)":dbl, "Error_Angulo_rad"=→"Error angular (rad)":dbl)  [unwired: 2 out]
    "Velocidad_Izq_m_s" <- w97
    "Velocidad_Der_m_s" <- w96
    "Distancia_Recorrida_m" <- w111
    "POSICIÓN X" <- w25
    "POSICIÓN Y" <- w24
    "PWM_Aplicado_Izq_pct" <- w94
    "PWM_Aplicado_Der_pct" <- w93
    "ORIENTACIÓN" <- w113
    n41 = Build Array (concatenate)(w92, w25) -> (w90:dbl[])
    n42 = xnode "PWM"("Duty Cycle"=w122) -> ()  [unwired: 1 in, 1 out]
    n43 = xnode "PWM"("Duty Cycle"=w123) -> ()  [unwired: 1 in, 1 out]
    n44 = Not Equal To 0?(x=w121) -> (x != 0?=w120:bool)
    n45 = Not Equal To 0?(x=w119) -> (x != 0?=w105:bool)
    n46 = Not Equal To 0?(x=w107) -> (x != 0?=→"Objetivo Alcanzado":bool)
    n47 = Bundle("Vel_Izq"=w97, "Vel_Der"=w96) -> (→"Grafica_Velocidades_m_s":cluster{"Vel_Izq":dbl, "Vel_Der":dbl})  [unwired: 1 in]
    n48 = xnode "Digital output (1 sample)"("B/DIO0 (Pin 11)"=w120) -> ()  [unwired: 1 in, 1 out]
    n49 = xnode "Digital output (1 sample)"("A/DIO0 (Pin 11)"=w105) -> ()  [unwired: 1 in, 1 out]
    n50 = Build Array (concatenate)(w91, w24) -> (w89:dbl[])
    n51 = Select(t=dbl[] [], s="RESET_TRAYECTO", f=w90) -> (s? t:f=w86:dbl[])
    n52 = Bundle("PWM_Final_Izq_pct"=w94, "PWM_Final_Der_pct"=w93) -> (→"Grafica_PWM_pct":T3)  [unwired: 1 in]
    n53 = Select(t=dbl[] [], s="RESET_TRAYECTO", f=w89) -> (s? t:f=w85:dbl[])
    n54 = Bundle("t"=w86, "t"=w85) -> (→"Grafica_Trayectoria_XY":cluster{"t":dbl[], "t":dbl[]})  [unwired: 1 in]
    n55 = Not Equal?(x=w77, y=T2."NINGUNA") -> (x != y?=w70:bool)
    n56 = And(x="Iniciar_Secuencia", y=w70) -> (x .and. y?=w69:bool)
    n57 = case shown="\"MOVER\"" w72 {
      tunnel: w69 -> [w264 _ _ _ _ _ _ _]
      tunnel: [w261 T4."MOVER" w268 T4."COMPROBAR_LLEGADA" T4."SIGUIENTE_TRAMO" w281 T4."FALLO" T4."FIN"] -> w57
      tunnel: "Finalizar tramo (simulación)" -> [_ _ w269 _ _ _ _ _]
      tunnel: w67 -> [_ w265 w267 w272 w274 w278 w286 w288]
      tunnel: [1 w265 w267 w272 w274 w276 w286 w288] -> w54
      frame "ESPERA", Default {
        n58 = Select(t=T4."PREPARAR_TRAMO", s=w264, f=T4."ESPERA") -> (s? t:f=w261:T4)
      }
      frame "PREPARAR_TRAMO" {
      }
      frame "MOVER" {
        n59 = Select(t=T4."FRENAR", s=w269, f=T4."MOVER") -> (s? t:f=w268:T4)
      }
      frame "FRENAR" {
      }
      frame "COMPROBAR_LLEGADA" {
      }
      frame "SIGUIENTE_TRAMO" {
        n60 = Less?(x=w278, y=3) -> (x < y?=w277:bool)
        n61 = Add(x=w278, y=1) -> (x+y=w279:i32)
        n62 = Select(t=T4."PREPARAR_TRAMO", s=w277, f=T4."FIN") -> (s? t:f=w281:T4)
        n63 = Select(t=w279, s=w277, f=w278) -> (s? t:f=w276:i32)
      }
      frame "FALLO" {
      }
      frame "FIN" {
      }
    }
    "Tramo Actual" <- w54
    "Estado de máquina" <- w57
    n64 = Subtract(x=w54, y=1) -> (x-y=w65:i32)
    n65 = Multiply(x=w65, y=33.333333333333) -> (x*y=w60:dbl)
    n66 = Select(t="SECUENCIA CARGADA", s=w70, f="EN ESPERA") -> (s? t:f=→"Estado de Operacion":string)
    n67 = Equal?(x=w57, y=T4."FIN") -> (x = y?=w62:bool)
    n68 = Select(t=100.0, s=w62, f=w60) -> (s? t:f=→"PROGRESO DE SECUENCIA":dbl)
    n69 = Select(t=T4."ESPERA" ("y"), s="Reiniciar_Ejecucion", f=w57) -> (s? t:f=w56:T4)
    n70 = Merge Signals(w25, w24) -> (w23:dynamicdata)
    n71 = xnode "Set Dynamic Data Attributes"("Signals In"=w23, "Signal Index"=0, "Signal Name"="X movil", "Unit"="m") -> ("Signals Out"=w22:dynamicdata)  [unwired: 1 in, 1 out]
    n72 = xnode "Set Dynamic Data Attributes"("Signals In"=w22, "Signal Index"=1, "Signal Name"="Y movil", "Unit"="m") -> ("Signals Out"=w21:dynamicdata)  [unwired: 1 in, 1 out]
    n73 = call "Write To Measurement File"("Signals"=w21) -> ()  [unwired: 16 in, 3 out]
  }
